vi "teststand epoch.vi"() -> (3 "time stamp":timestamp)   [LabVIEW 2020, in "nominal teststand model sequence support.lvlib"]
uses:
  nominal teststand model sequence support.lvlib
  <vilib>/Utility/miscctls.llb/LVDateTimeRec.ctl
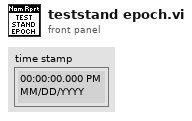
[diagram p1: front panel]
types:
  T1 = typedef "LVDateTimeRec.ctl" = cluster{"fractional second":dbl, "second":i32, "minute":i32, "hour":i32, "day of month":i32, "month":i32, "year":i32, "day of week":i32, "day of year":i32, "DST":i32}
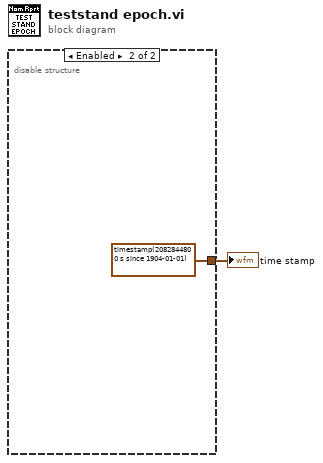
[diagram p0: block diagram]
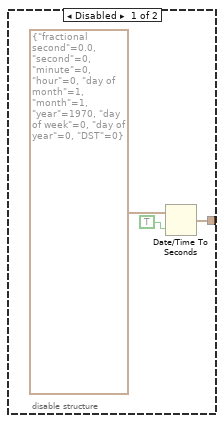
[diagram p2: hidden frame]
diagram:
  n1 = disable-structure shown="Enabled" {
    disable-tunnel: [w4 timestamp(2082844800 s since 1904-01-01) ("time stamp")] -> w1
    frame Disabled {
      n2 = Date/Time To Seconds(1:TRUE ("is UTC (F)"), 2:T1 {"fractional second"=0.0, "second"=0, "minute"=0, "hour"=0, "day of month"=1, "month"=1, "year"=1970, "day of week"=0, "day of year"=0, "DST"=0} ("date time rec")) -> (0:w4:timestamp)
    }
    frame Enabled {
    }
  }
  "time stamp" <- w1
